vi "RemoteVI Write To Clients.vi"(0 "clients":T1(array[cluster]), 5 "data":string, 7 "timeout ms":i32=500) -> (4 "clients out":T1(array[cluster]))   [LabVIEW 2020, in "RemoteVI.lvlib"]
doc: "Writes data (a complete WebSocket frame) to every client that is not closed, with timeout ms per client; a client whose write fails is marked closed. Connections are TCP refnums type-cast to U32."
uses:
  RemoteVI.lvlib
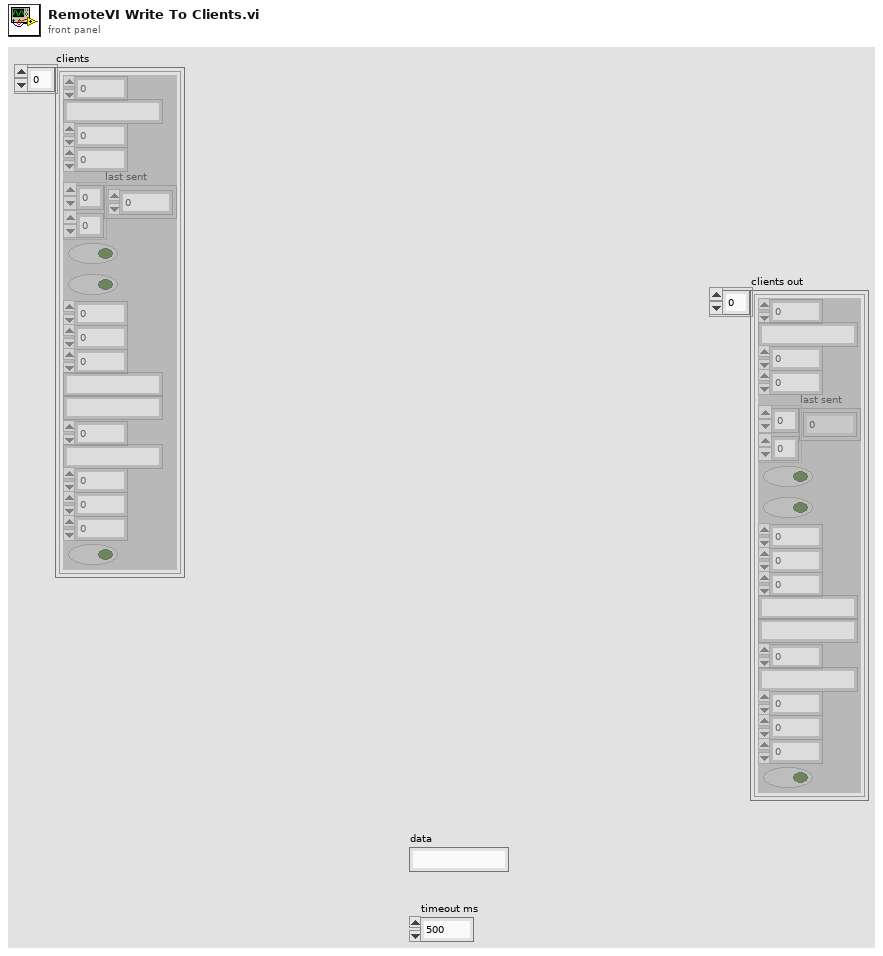
[diagram p1: front panel]
types:
  T1 = cluster{"connection":u32, "rx buffer":string, "seq":u32, "acked":u32, "last sent":u32[][], "tracking":bool, "closed":bool, "mods":u8, "mods set":u8, "popup since":u32, "windows sent":string, "window frames":cluster{"id":u64, "pixels":u32[][]}[], "key window":u64, "address":string, "since":dbl, "last input":dbl, "bytes":dbl, "view only":bool}[]
  T2 = cluster{"connection":u32, "rx buffer":string, "seq":u32, "acked":u32, "last sent":u32[][], "tracking":bool, "closed":bool, "mods":u8, "mods set":u8, "popup since":u32, "windows sent":string, "window frames":cluster{"id":u64, "pixels":u32[][]}[], "key window":u64, "address":string, "since":dbl, "last input":dbl, "bytes":dbl, "view only":bool}
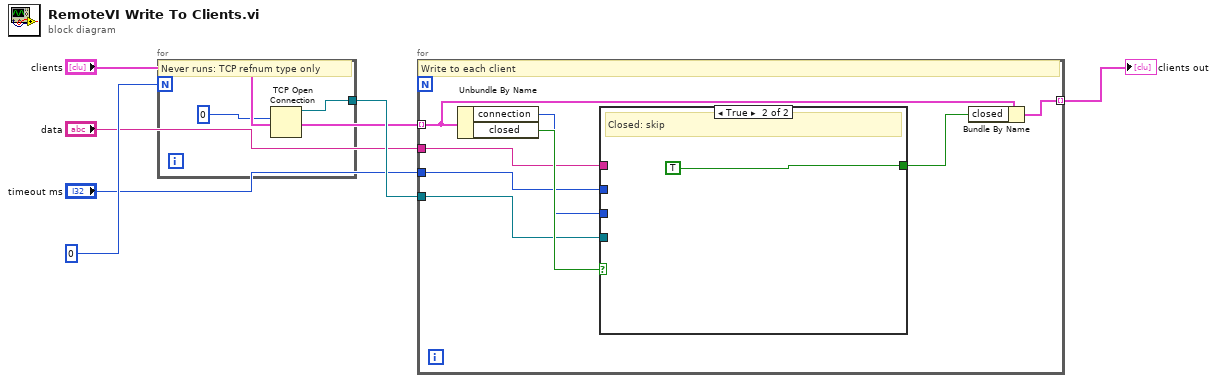
[diagram p0: block diagram]
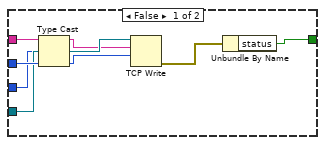
[diagram p2: hidden frame]
diagram:
  n1 = for {
    N: 0 -> [_]
    tunnel: [w8] -> w5
    # "Never runs: TCP refnum type only"
    n2 = TCP Open Connection(remote port or service name=u16 0) -> (connection ID=w8:refnum<k5>)  [unwired: 4 in, 1 out]
  }
  n3 = for {
    tunnel: "clients" -> [w9] mode=indexing
    tunnel: "data" -> [w10]
    tunnel: "timeout ms" -> [w12]
    tunnel: w5 -> [w11]
    tunnel: [w16] -> w6 mode=indexing
    # "Write to each client"
    n4 = Unbundle By Name(w9) -> ("connection"=w13:u32, "closed"=w14:bool)
    n5 = case shown="True" w14 {
      tunnel: [w23 TRUE] -> w15
      tunnel: w10 -> [w18 _]
      tunnel: w12 -> [w20 _]
      tunnel: w13 -> [w17 _]
      tunnel: w11 -> [w19 _]
      frame False {
        n6 = Type Cast(type=w19, x=w17) -> (*(type *) &x=w21:refnum<k5>)
        n7 = TCP Write(connection ID=w21, data in=w18, 9:w20) -> (error out=w22:errorcluster)  [unwired: 1 in, 2 out]
        n8 = Unbundle By Name(w22) -> ("status"=w23:bool)
      }
      frame True {
        # "Closed: skip"
      }
    }
    n9 = Bundle By Name(cluster=w9, "closed"=w15) -> (w16:T2)
  }
  "clients out" <- w6
